vi "current calibration.vi"(11 "Current":dbl format="%#_13g") -> (3 "CURRENT mA":dbl)   [LabVIEW 2026]
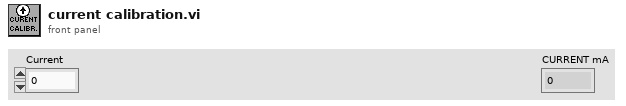
[diagram p1: front panel]
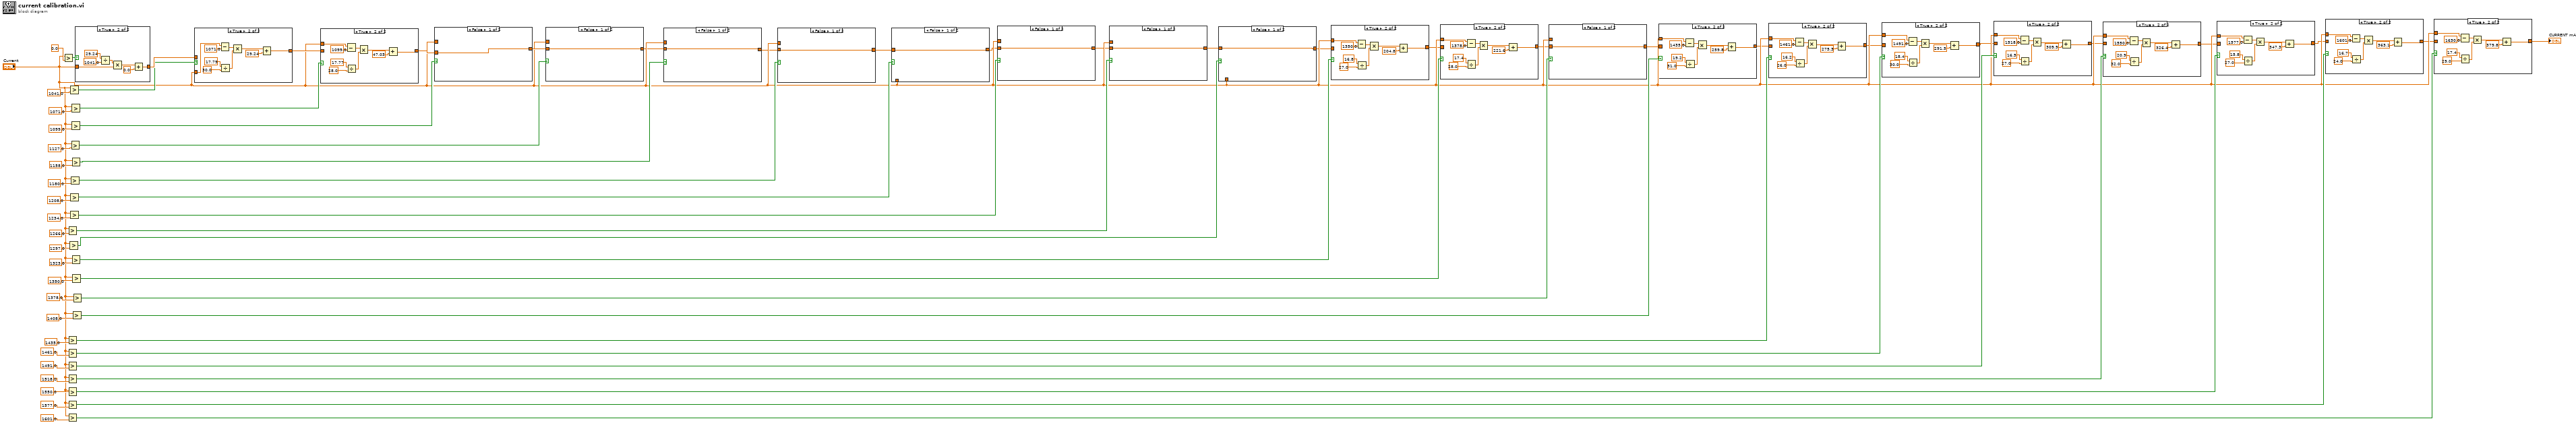
[diagram p0: block diagram]
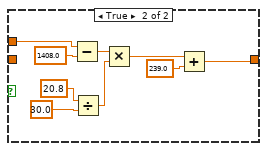
[diagram p10: hidden frame]
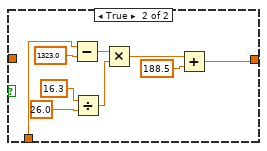
[diagram p13: hidden frame]
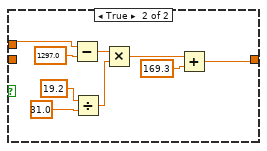
[diagram p14: hidden frame]
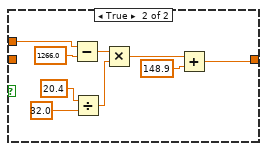
[diagram p15: hidden frame]
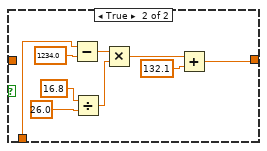
[diagram p16: hidden frame]
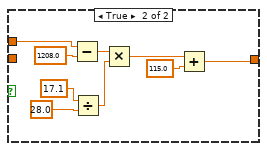
[diagram p17: hidden frame]
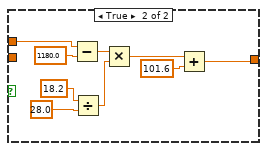
[diagram p18: hidden frame]
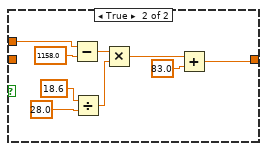
[diagram p19: hidden frame]
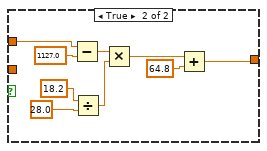
[diagram p20: hidden frame]
diagram:
  n1 = Greater?(x="Current", y=0.0) -> (0:w66:bool)
  n2 = Greater?(x="Current", y=1266.0) -> (0:w42:bool)
  n3 = Greater?(x="Current", y=1435.0) -> (0:w33:bool)
  n4 = Greater?(x="Current", y=1461.0) -> (0:w31:bool)
  n5 = Greater?(x="Current", y=1491.0) -> (0:w28:bool)
  n6 = Greater?(x="Current", y=1518.0) -> (0:w26:bool)
  n7 = Greater?(x="Current", y=1550.0) -> (0:w24:bool)
  n8 = Greater?(x="Current", y=1577.0) -> (0:w23:bool)
  n9 = Greater?(x="Current", y=1601.0) -> (0:w20:bool)
  n10 = Greater?(x="Current", y=1297.0) -> (0:w41:bool)
  n11 = Greater?(x="Current", y=1041.0) -> (0:w63:bool)
  n12 = Greater?(x="Current", y=1208.0) -> (0:w44:bool)
  n13 = Greater?(x="Current", y=1234.0) -> (0:w43:bool)
  n14 = Greater?(x="Current", y=1180.0) -> (0:w45:bool)
  n15 = Greater?(x="Current", y=1127.0) -> (0:w55:bool)
  n16 = Greater?(x="Current", y=1071.0) -> (0:w58:bool)
  n17 = Greater?(x="Current", y=1099.0) -> (0:w56:bool)
  n18 = Greater?(x="Current", y=1158.0) -> (0:w54:bool)
  n19 = Greater?(x="Current", y=1323.0) -> (0:w40:bool)
  n20 = Greater?(x="Current", y=1350.0) -> (0:w38:bool)
  n21 = Greater?(x="Current", y=1408.0) -> (0:w34:bool)
  n22 = Greater?(x="Current", y=1378.0) -> (0:w36:bool)
  n23 = case shown="True" w66 {
    tunnel: [0.0 w70] -> w65
    tunnel: "Current" -> [_ w69]
    frame False {
    }
    frame True {
      n24 = Divide(x=29.24 ("y"), y=1041.0) -> (x/y=w75:dbl)
      n25 = Multiply(x=w75, y=w69) -> (x*y=w71:dbl)
      n26 = Add(x=w71, y=0.0 ("x")) -> (x+y=w70:dbl)
    }
  }
  n27 = case shown="True" w63 {
    tunnel: w65 -> [w76 _]
    tunnel: "Current" -> [_ w85]
    tunnel: [w76 w77] -> w57
    frame False {
    }
    frame True {
      n28 = Subtract(x=w85, y=1071.0) -> (x-y=w83:dbl)
      n29 = Divide(x=17.79, y=30.0) -> (x/y=w82:dbl)
      n30 = Multiply(x=w83, y=w82) -> (x*y=w81:dbl)
      n31 = Add(x=w81, y=29.24) -> (x+y=w77:dbl)
    }
  }
  n32 = case shown="True" w58 {
    tunnel: "Current" -> [_ w88]
    tunnel: w57 -> [w86 _]
    tunnel: [w86 w87] -> w53
    frame False {
    }
    frame True {
      n33 = Subtract(x=w88, y=1099.0) -> (x-y=w94:dbl)
      n34 = Divide(x=17.77, y=28.0) -> (x/y=w93:dbl)
      n35 = Multiply(x=w94, y=w93) -> (x*y=w92:dbl)
      n36 = Add(x=w92, y=47.03) -> (x+y=w87:dbl)
    }
  }
  n37 = case shown="False" w56 {
    tunnel: "Current" -> [_ w98]
    tunnel: [w96 w97] -> w52
    tunnel: w53 -> [w96 _]
    frame False {
    }
    frame True {
      n38 = Subtract(x=w98, y=1127.0) -> (x-y=w104:dbl)
      n39 = Divide(x=18.2, y=28.0) -> (x/y=w103:dbl)
      n40 = Multiply(x=w104, y=w103) -> (x*y=w102:dbl)
      n41 = Add(x=w102, y=64.8) -> (x+y=w97:dbl)
    }
  }
  n42 = case shown="False" w55 {
    tunnel: "Current" -> [_ w108]
    tunnel: w52 -> [w106 _]
    tunnel: [w106 w107] -> w18
    frame False {
    }
    frame True {
      n43 = Subtract(x=w108, y=1158.0) -> (x-y=w114:dbl)
      n44 = Divide(x=18.6, y=28.0) -> (x/y=w113:dbl)
      n45 = Multiply(x=w114, y=w113) -> (x*y=w112:dbl)
      n46 = Add(x=w112, y=83.0) -> (x+y=w107:dbl)
    }
  }
  n47 = case shown="False" w54 {
    tunnel: "Current" -> [_ w118]
    tunnel: [w116 w117] -> w17
    tunnel: w18 -> [w116 _]
    frame False {
    }
    frame True {
      n48 = Subtract(x=w118, y=1180.0) -> (x-y=w124:dbl)
      n49 = Divide(x=18.2, y=28.0) -> (x/y=w123:dbl)
      n50 = Multiply(x=w124, y=w123) -> (x*y=w122:dbl)
      n51 = Add(x=w122, y=101.6) -> (x+y=w117:dbl)
    }
  }
  n52 = case shown="False" w45 {
    tunnel: [w126 w128] -> w16
    tunnel: "Current" -> [_ w127]
    tunnel: w17 -> [w126 _]
    frame False {
    }
    frame True {
      n53 = Subtract(x=w127, y=1208.0) -> (x-y=w134:dbl)
      n54 = Divide(x=17.1, y=28.0) -> (x/y=w133:dbl)
      n55 = Multiply(x=w134, y=w133) -> (x*y=w132:dbl)
      n56 = Add(x=w132, y=115.0) -> (x+y=w128:dbl)
    }
  }
  n57 = case shown="False" w44 {
    tunnel: [w136 w138] -> w15
    tunnel: "Current" -> [_ w137]
    tunnel: w16 -> [w136 _]
    frame False {
    }
    frame True {
      n58 = Subtract(x=w137, y=1234.0) -> (x-y=w144:dbl)
      n59 = Divide(x=16.8, y=26.0) -> (x/y=w143:dbl)
      n60 = Multiply(x=w144, y=w143) -> (x*y=w142:dbl)
      n61 = Add(x=w142, y=132.1) -> (x+y=w138:dbl)
    }
  }
  n62 = case shown="False" w43 {
    tunnel: [w146 w148] -> w14
    tunnel: "Current" -> [_ w147]
    tunnel: w15 -> [w146 _]
    frame False {
    }
    frame True {
      n63 = Subtract(x=w147, y=1266.0) -> (x-y=w154:dbl)
      n64 = Divide(x=20.4, y=32.0) -> (x/y=w153:dbl)
      n65 = Multiply(x=w154, y=w153) -> (x*y=w152:dbl)
      n66 = Add(x=w152, y=148.9) -> (x+y=w148:dbl)
    }
  }
  n67 = case shown="False" w42 {
    tunnel: [w156 w158] -> w13
    tunnel: "Current" -> [_ w157]
    tunnel: w14 -> [w156 _]
    frame False {
    }
    frame True {
      n68 = Subtract(x=w157, y=1297.0) -> (x-y=w164:dbl)
      n69 = Divide(x=19.2, y=31.0) -> (x/y=w163:dbl)
      n70 = Multiply(x=w164, y=w163) -> (x*y=w162:dbl)
      n71 = Add(x=w162, y=169.3) -> (x+y=w158:dbl)
    }
  }
  n72 = case shown="False" w41 {
    tunnel: [w166 w168] -> w12
    tunnel: "Current" -> [_ w167]
    tunnel: w13 -> [w166 _]
    frame False {
    }
    frame True {
      n73 = Subtract(x=w167, y=1323.0) -> (x-y=w174:dbl)
      n74 = Divide(x=16.3, y=26.0) -> (x/y=w173:dbl)
      n75 = Multiply(x=w174, y=w173) -> (x*y=w172:dbl)
      n76 = Add(x=w172, y=188.5) -> (x+y=w168:dbl)
    }
  }
  n77 = case shown="True" w40 {
    tunnel: [w176 w178] -> w11
    tunnel: "Current" -> [_ w177]
    tunnel: w12 -> [w176 _]
    frame False {
    }
    frame True {
      n78 = Subtract(x=w177, y=1350.0) -> (x-y=w184:dbl)
      n79 = Divide(x=16.8, y=27.0) -> (x/y=w183:dbl)
      n80 = Multiply(x=w184, y=w183) -> (x*y=w182:dbl)
      n81 = Add(x=w182, y=204.8) -> (x+y=w178:dbl)
    }
  }
  n82 = case shown="True" w38 {
    tunnel: [w186 w188] -> w10
    tunnel: "Current" -> [_ w187]
    tunnel: w11 -> [w186 _]
    frame False {
    }
    frame True {
      n83 = Subtract(x=w187, y=1378.0) -> (x-y=w194:dbl)
      n84 = Divide(x=17.4, y=28.0) -> (x/y=w193:dbl)
      n85 = Multiply(x=w194, y=w193) -> (x*y=w192:dbl)
      n86 = Add(x=w192, y=221.6) -> (x+y=w188:dbl)
    }
  }
  n87 = case shown="False" w36 {
    tunnel: [w196 w198] -> w9
    tunnel: "Current" -> [_ w197]
    tunnel: w10 -> [w196 _]
    frame False {
    }
    frame True {
      n88 = Subtract(x=w197, y=1408.0) -> (x-y=w204:dbl)
      n89 = Divide(x=20.8, y=30.0) -> (x/y=w203:dbl)
      n90 = Multiply(x=w204, y=w203) -> (x*y=w202:dbl)
      n91 = Add(x=w202, y=239.0) -> (x+y=w198:dbl)
    }
  }
  n92 = case shown="True" w34 {
    tunnel: [w206 w208] -> w8
    tunnel: "Current" -> [_ w207]
    tunnel: w9 -> [w206 _]
    frame False {
    }
    frame True {
      n93 = Subtract(x=w207, y=1435.0) -> (x-y=w214:dbl)
      n94 = Divide(x=19.2, y=31.0) -> (x/y=w213:dbl)
      n95 = Multiply(x=w214, y=w213) -> (x*y=w212:dbl)
      n96 = Add(x=w212, y=259.8) -> (x+y=w208:dbl)
    }
  }
  n97 = case shown="True" w33 {
    tunnel: [w216 w218] -> w7
    tunnel: "Current" -> [_ w217]
    tunnel: w8 -> [w216 _]
    frame False {
    }
    frame True {
      n98 = Subtract(x=w217, y=1461.0) -> (x-y=w224:dbl)
      n99 = Divide(x=16.2, y=26.0) -> (x/y=w223:dbl)
      n100 = Multiply(x=w224, y=w223) -> (x*y=w222:dbl)
      n101 = Add(x=w222, y=275.3) -> (x+y=w218:dbl)
    }
  }
  n102 = case shown="True" w31 {
    tunnel: [w226 w228] -> w6
    tunnel: "Current" -> [_ w227]
    tunnel: w7 -> [w226 _]
    frame False {
    }
    frame True {
      n103 = Subtract(x=w227, y=1491.0) -> (x-y=w234:dbl)
      n104 = Divide(x=18.4, y=30.0) -> (x/y=w233:dbl)
      n105 = Multiply(x=w234, y=w233) -> (x*y=w232:dbl)
      n106 = Add(x=w232, y=291.5) -> (x+y=w228:dbl)
    }
  }
  n107 = case shown="True" w28 {
    tunnel: [w236 w238] -> w5
    tunnel: "Current" -> [_ w237]
    tunnel: w6 -> [w236 _]
    frame False {
    }
    frame True {
      n108 = Subtract(x=w237, y=1518.0) -> (x-y=w244:dbl)
      n109 = Divide(x=16.5, y=27.0) -> (x/y=w243:dbl)
      n110 = Multiply(x=w244, y=w243) -> (x*y=w242:dbl)
      n111 = Add(x=w242, y=309.9) -> (x+y=w238:dbl)
    }
  }
  n112 = case shown="True" w26 {
    tunnel: [w246 w248] -> w4
    tunnel: "Current" -> [_ w247]
    tunnel: w5 -> [w246 _]
    frame False {
    }
    frame True {
      n113 = Subtract(x=w247, y=1550.0) -> (x-y=w254:dbl)
      n114 = Divide(x=20.9, y=32.0) -> (x/y=w253:dbl)
      n115 = Multiply(x=w254, y=w253) -> (x*y=w252:dbl)
      n116 = Add(x=w252, y=326.4) -> (x+y=w248:dbl)
    }
  }
  n117 = case shown="True" w24 {
    tunnel: [w256 w258] -> w3
    tunnel: "Current" -> [_ w257]
    tunnel: w4 -> [w256 _]
    frame False {
    }
    frame True {
      n118 = Subtract(x=w257, y=1577.0) -> (x-y=w264:dbl)
      n119 = Divide(x=15.8, y=27.0) -> (x/y=w263:dbl)
      n120 = Multiply(x=w264, y=w263) -> (x*y=w262:dbl)
      n121 = Add(x=w262, y=347.3) -> (x+y=w258:dbl)
    }
  }
  n122 = case shown="True" w23 {
    tunnel: [w266 w268] -> w2
    tunnel: "Current" -> [_ w267]
    tunnel: w3 -> [w266 _]
    frame False {
    }
    frame True {
      n123 = Subtract(x=w267, y=1601.0) -> (x-y=w274:dbl)
      n124 = Divide(x=16.7, y=24.0) -> (x/y=w273:dbl)
      n125 = Multiply(x=w274, y=w273) -> (x*y=w272:dbl)
      n126 = Add(x=w272, y=363.1) -> (x+y=w268:dbl)
    }
  }
  n127 = case shown="True" w20 {
    tunnel: [w276 w278] -> w1
    tunnel: "Current" -> [_ w277]
    tunnel: w2 -> [w276 _]
    frame False {
    }
    frame True {
      n128 = Subtract(x=w277, y=1630.0) -> (x-y=w284:dbl)
      n129 = Divide(x=17.4, y=29.0) -> (x/y=w283:dbl)
      n130 = Multiply(x=w284, y=w283) -> (x*y=w282:dbl)
      n131 = Add(x=w282, y=379.8) -> (x+y=w278:dbl)
    }
  }
  "CURRENT mA" <- w1
